vi "Seq_list_load.vi"(8 "error in":errorcluster) -> (0 "error out":errorcluster, 2 "selected Seq":string[](array[string]), 3 "selected sample name":string[](array[string]))   [LabVIEW 2018]
panel:
  out "array 2":string[][](array[string])
  out "stripped path":path
  in  "Set":bool
  in  "Receip Name":u16(ring) items=["Amino_peptide2_Data.csv", "Amino_peptide_Data.csv", "Baseset.csv", "CpG_20221102.csv", "Hashimoto_poly.csv", "Hashimoto_Var.csv", "Hitachi_20260113.csv", "HU.csv", "Kumamoto2nd_20221104.csv", "Kumamoto3nd_20230118_KSTKSN_m.csv", "Kumamoto4nd_20230119_KSTKSN_m.csv", "Kumamoto_20221104.csv", "kumamoto_NSVR_20231019.csv", "kumamoto_NSVR_20260901.csv", "LENK_AENK.csv", "Mitsuzawa_001.csv", "Neoantigen_Data_01.csv", "Neoantigen_Data_02.csv", "Neoantigen_Data_03.csv", "Neoantigen_Data_04.csv", "Neoantigen_Data_05.csv", "Neoantigen_Data_06.csv", "Neoantigen_Data_07.csv", "Neoantigen_Data_237.csv", "Neoantigen_Data_272.csv", "Neoantigen_Data_374.csv", "Neoantigen_Data_380.csv", "Neoantigen_Data_HCT116.csv", "Neoantigen_Data_XX.csv", "Neoantigen_Epi_Data_01.csv", "Neoantigen_Epi_Data_01_for cell line.csv", "Neoantigen_EpiPhos_380_20250915.csv", "Neoantigen_EpiPhos_HCT117_01.csv", "Neoantigen_EpiPhos_HCT117_20250915.csv", "NPR1_m6A_20221104.csv", "Pac_miRNA_01.csv", "PhiX.csv", "PhiX2.csv", "Ploop_Data.csv", "Sakano_vaso_20260906.csv", "SEQ Data.csv", "Takahagi_13fix.csv", "Takahagi_13fix_DNARNA.csv", "Takahagi_13fix_pep.csv", "Takahagi_LaTNA.csv", "Takahagi_Xen17.csv", "Takahagi_Xeno.csv", "Takahagi_zeno12.csv", "U_methyl.csv", "VHH_variant_20231020_115356_sq_list.csv", "VHH_variant_20231026_115356_sq_list.csv"]
  out "appended path":path
  out "ACond#":i32
  in  "index":i32
  out "Array 2":string[](array[string])
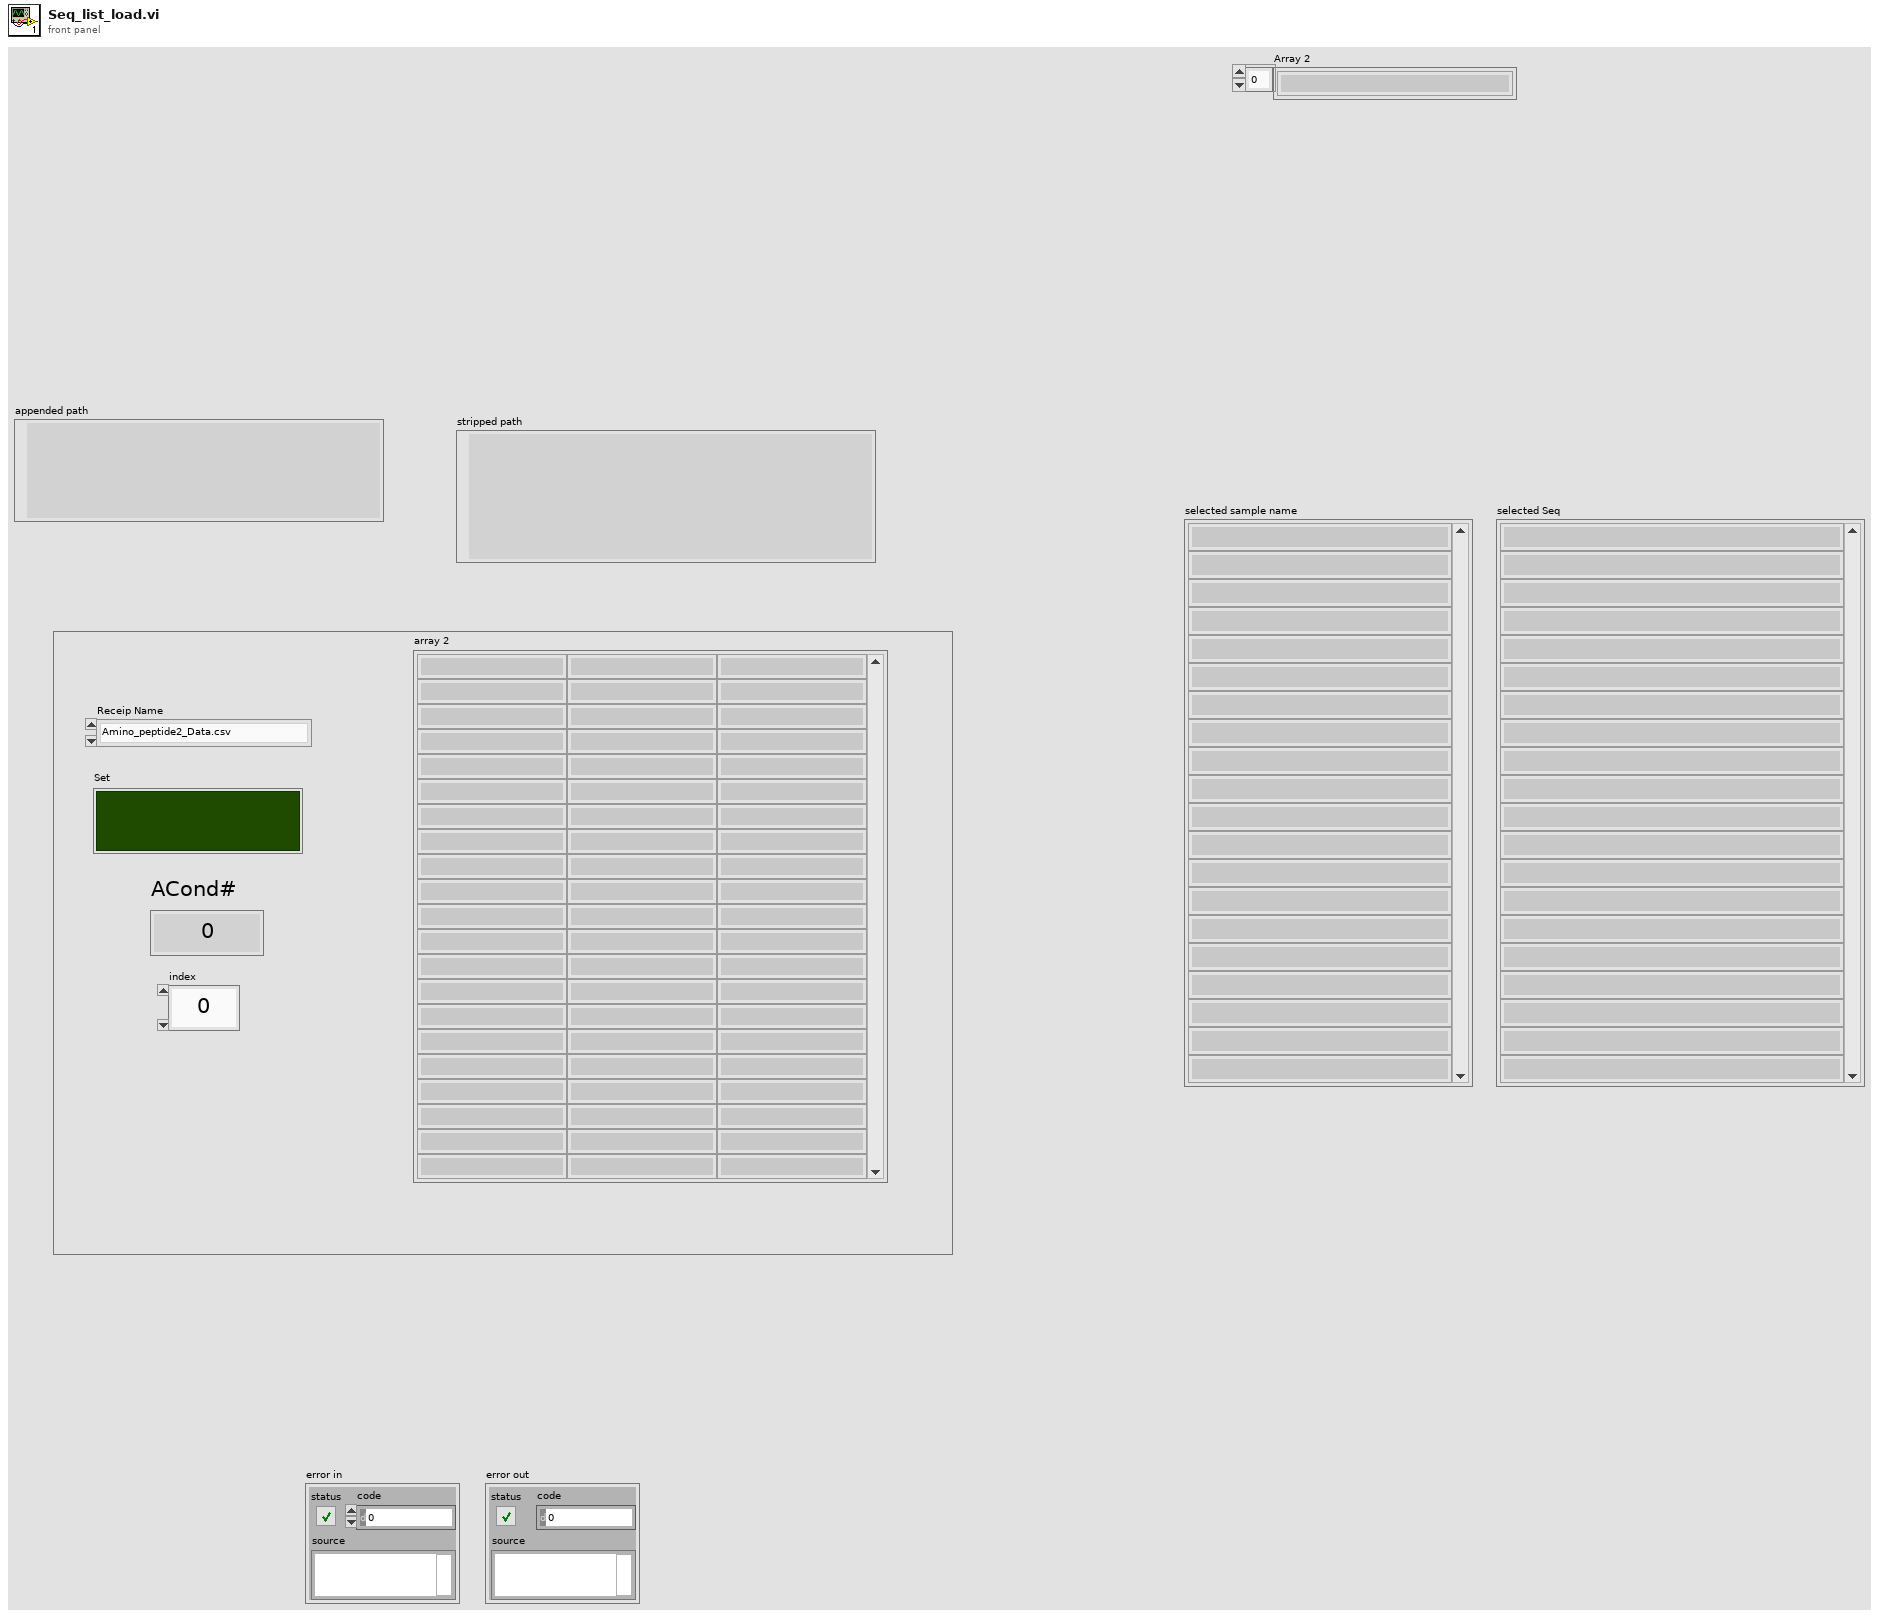
[diagram p1: front panel]
types:
  T1 = enum16{"open", "replace", "create", "open or create", "replace or create", "replace or create with confirmation"}
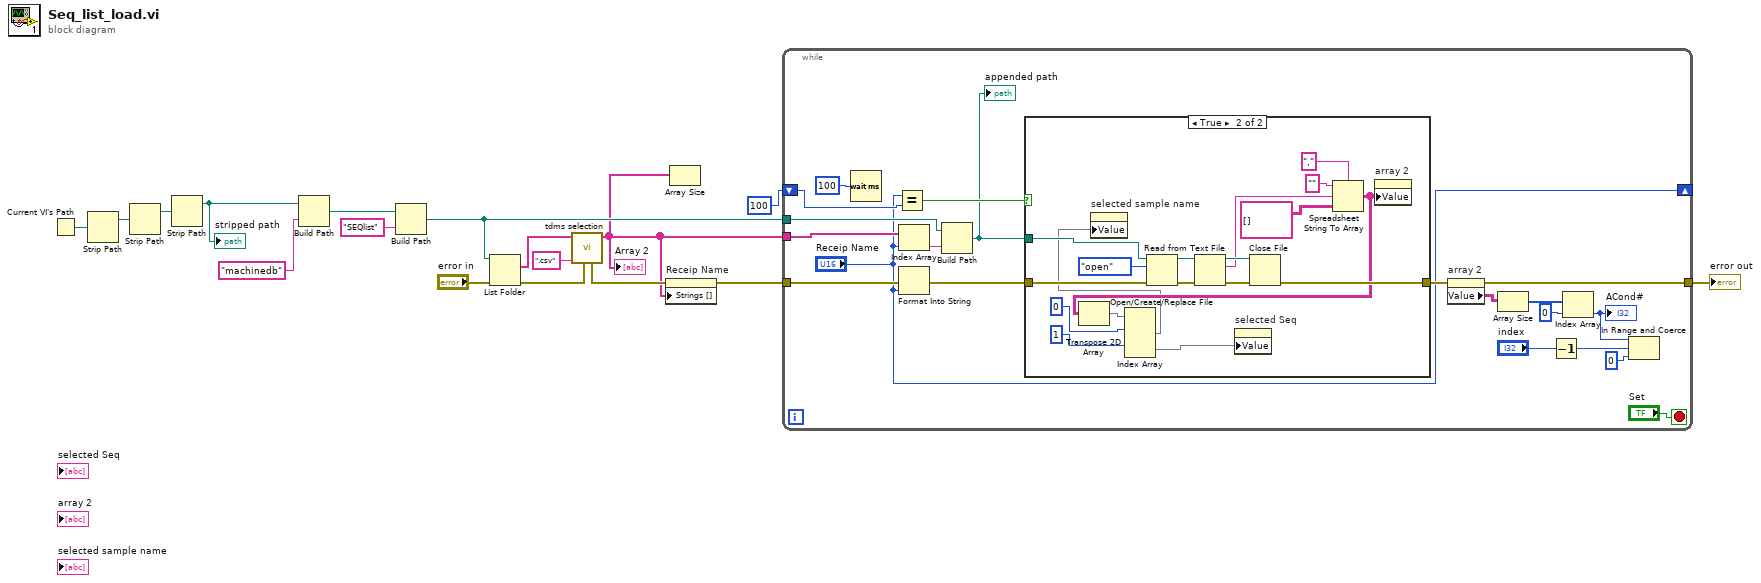
[diagram p0: block diagram]
diagram:
  n1 = Current VI's Path() -> (path=w10:path)
  n2 = Strip Path(path=w10) -> (stripped path=w9:path)  [unwired: 1 out]
  n3 = Strip Path(path=w9) -> (stripped path=w8:path)  [unwired: 1 out]
  n4 = Strip Path(path=w8) -> (stripped path=w7:path)  [unwired: 1 out]
  "stripped path" <- w7
  n5 = Build Path(base path=w7, name or relative path="machinedb") -> (appended path=w5:path)
  n6 = Build Path(base path=w5, name or relative path="SEQlist") -> (appended path=w3:path)
  n7 = List Folder(path=w3, error in="error in") -> (filenames=w17:string[], error out=w15:errorcluster)  [unwired: 2 in, 2 out]
  n8 = call "tdms selection.vi"("error in"=w15, "string"=".csv", "Filename List"=w17) -> ("Array 2"=w1:string[], "error out"=w12:errorcluster)  [unwired: 6 in, 1 out]
  "Array 2" <- w1
  n9 = property on="Receip Name" class="Ring (strict)"(error in=w12, "Strings []"=w1) -> (error out=w11:errorcluster)  [unwired: 1 in, 1 out]
  n10 = Array Size(array=w1) -> ()  [unwired: 1 out]
  n11 = while {
    tunnel: w11 -> [w36]
    tunnel: [w21] -> w13
    tunnel: w3 -> [w35]
    tunnel: w1 -> [w33]
    shift-right: ["Receip Name"] -> _
    shift-left: u16 100 ("Receip Name") -> [w19]
    stop <- "Set" stop-if-true
    n12 = Wait (ms)(milliseconds to wait=u32 100) -> ()  [unwired: 1 out]
    n13 = Equal?(x="Receip Name", y=w19) -> (x = y?=w31:bool)
    n14 = Index Array(array=w33, index="Receip Name") -> (element=w32:string)
    n15 = Format Into String(error in=w36, "Receip Name") -> (error out=w30:errorcluster)  [unwired: 2 in, 1 out]
    n16 = Build Path(base path=w35, name or relative path=w32) -> (appended path=w29:path)
    "appended path" <- w29
    n17 = case shown="True" w31 {
      tunnel: w30 -> [w38 w54]
      tunnel: [w38 w51] -> w22
      tunnel: w29 -> [_ w56]
      frame False {
      }
      frame True {
        n18 = Open/Create/Replace File(file path (use dialog)=w56, error in=w54, operation (0:open)=T1."open") -> (refnum out=w50:refnum<file>, error out=w53:errorcluster)  [unwired: 3 in, 1 out]
        n19 = Read from Text File(file (use dialog)=w50, error in=w53) -> (refnum out=w49:refnum<file>, text=w48:string, error out=w52:errorcluster)  [unwired: 2 in, 1 out]
        n20 = Close File(refnum=w49, error in=w52) -> (error out=w51:errorcluster)  [unwired: 1 out]
        n21 = Spreadsheet String To Array(delimiter (Tab)=",", format string="", spreadsheet string=w48, array type (2D Dbl)=string[][] [] ("delimiter (Tab)")) -> (array=w41:string[][])
        n22 = Transpose 2D Array(2D array=w41) -> (transposed array=w44:string[][])
        n23 = Index Array(array=w44, index (row) #1=0 ("index (row)"), index (row) #2=1 ("index (row)")) -> (element #1=w40:string[], element #2=w39:string[])  [unwired: 2 in]
        n24 = property on="selected sample name" class="Arr (strict)"("Value"=w40) -> ()  [unwired: 2 in, 2 out]
        n25 = property on="selected Seq" class="Arr (strict)"("Value"=w39) -> ()  [unwired: 2 in, 2 out]
        n26 = property on="array 2" class="Arr (strict)"("Value"=w41) -> ()  [unwired: 2 in, 2 out]
      }
    }
    n27 = property on="array 2" class="Arr (strict)"(error in=w22) -> (error out=w21:errorcluster, "Value"=w20:string[][])  [unwired: 1 in, 1 out]
    n28 = Array Size(array=w20) -> (size(s)=w25:i32[])
    n29 = Decrement(x="index") -> (x-1=w27:i32)
    n30 = Index Array(array=w25, index=0) -> (element=w23:i32)
    "ACond#" <- w23
    n31 = In Range and Coerce(upper limit=w23, x=w27, lower limit=0) -> ()  [unwired: 2 out]
  }
  "error out" <- w13
